vi "Stop Motor.vi"(8 "error in (no error)":errorcluster, 10 "Target":enum16{"Mast", "Turn Table"}(ring), 11 "AUDIX EM1000 in":refnum<class "AUDIX EM1000.lvclass">) -> (0 "error out":errorcluster, 3 "AUDIX EM1000 out":refnum<class "AUDIX EM1000.lvclass">)   [LabVIEW 2023, in "Turn Table and Mast.lvlib" / "AUDIX EM1000.lvclass"]
uses:
  AUDIX EM1000.lvclass
  AUDIX EM1000.lvclass/AUDIX EM1000.ctl
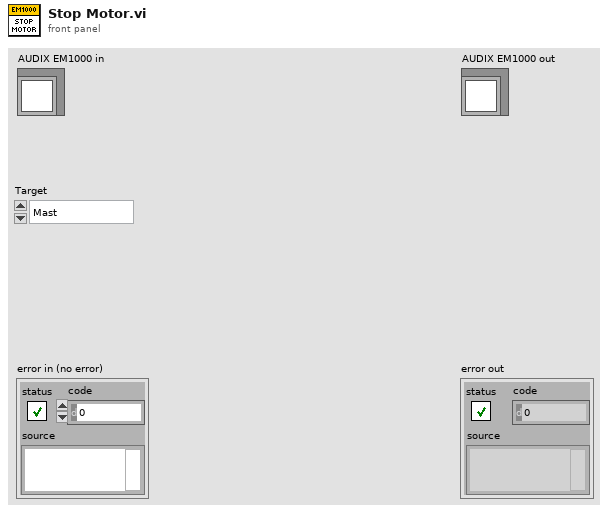
[diagram p1: front panel]
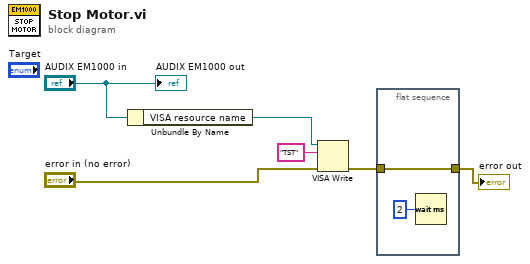
[diagram p0: block diagram]
diagram:
  n1 = Unbundle By Name("AUDIX EM1000 in") -> ("VISA resource name"=w4:refnum<visa-resource-name>)
  n2 = VISA Write(VISA resource name=w4, write buffer="TST" ("버퍼 쓰기"), error in (no error)="error in (no error)") -> (error out=w2:errorcluster)  [unwired: 2 out]
  n3 = flat-sequence {
    tunnel: w2 -> [w8]
    tunnel: [w8] -> w1
    frame #0 {
      n4 = Wait (ms)(milliseconds to wait=u32 2) -> ()  [unwired: 1 out]
    }
  }
  "error out" <- w1
  "AUDIX EM1000 out" <- "AUDIX EM1000 in"
